vi "Resolve Request State.vi"(7 "status code in":u16, 8 "error in":errorcluster, 9 "response in":string, 10 "refused in":bool, 11 "MCP Request Metadata":T1) -> (0 "error out":errorcluster, 1 "response":string, 2 "refused":bool, 3 "MCP Request Metadata out":T1, 5 "status code":u16)   [LabVIEW 2020, in "MCP Server.lvlib"]
doc: "Resolves the requestState of a modern request (MCP 2026-07-28, multi round-trip requests). Called by Handle MCP Request.vi after Check Modern MCP Request.vi and before Set MCP Request Context.vi, and by Prepare Request Dispatch.vi, so that a refused requestState is answered as a plain HTTP error and never streamed.\n\nWHY: the client sends back only the answers to the LATEST inputRequests, together with the opaque requestState token of the previous input_required result. The answers of the earlier rounds stay in the server (Request State Store.vi) and are merged in here, so a tool that asks several questions in several rounds (Ask User.vi) finds every answer it was given.\n\n- No requestState (request state of MCP Request Metadata.ctl empty), a legacy request, or a request already refused (refused in): everything is passed through unchanged.\n- requestState given: the token is taken from Request State Store.vi. It is refused when it is unknown or expired, or when the method, params.name or the arguments digest (SHA-256 of params.arguments, see Read MCP Request Metadata.vi) differ from the ones it was issued for: refused becomes TRUE, status code 400, response {\"jsonrpc\":\"2.0\",\"id\":<id>,\"error\":{\"code\":-32602,\"message\":\"Invalid params: requestState is unknown, expired or belongs to another request\"}}.\n- Found and matching: input responses of MCP Request Metadata out = the stored answers (\"answers\" of the stored state) merged with the request's inputResponses; the request's value wins for the same key, and keys the tool does not ask for are kept (Ask User.vi ignores them).\n\nThe JSONtext errors are merged and cleared here. error in is passed through unchanged and does not stop the resolution."
uses:
  MCP Server.lvlib
  MCP Request Metadata.ctl
  <vilib>/JDP Science/JSONtext/Next JSON Value.vi
  <vilib>/JDP Science/JSONtext/String Subset.vi
  <vilib>/JDP Science/JSONtext/Parsing/Advance past next JSON Value (inlined COPY).vi
  <vilib>/JDP Science/JSONtext/Parsing/Advance past whitespace.vi
  <vilib>/JDP Science/JSONtext/Parsing/Advance past String.vi
  <vilib>/JDP Science/JSONtext/Parsing/Advance past Number.vi
  <vilib>/JDP Science/JSONtext/Parsing/Advance past Line Ending.vi
  <vilib>/JDP Science/JSONtext/Parsing/Parse Full Path or Item Name.vi
  <vilib>/JDP Science/JSONtext/Parsing/Advance past Array.vi
  <vilib>/JDP Science/JSONtext/Parsing/Advance past Object.vi
  <vilib>/JDP Science/JSONtext/support/Error Cluster From Code.vi
  <vilib>/JDP Science/JSONtext/Offset/Find Item Locations by Path.vi
  <vilib>/JDP Science/JSONtext/Get all Object Items.vi
  <vilib>/JDP Science/JSONtext/Set Multiple Object Items.vi
  <vilib>/JDP Science/JSONtext/JSONtext.lvlib
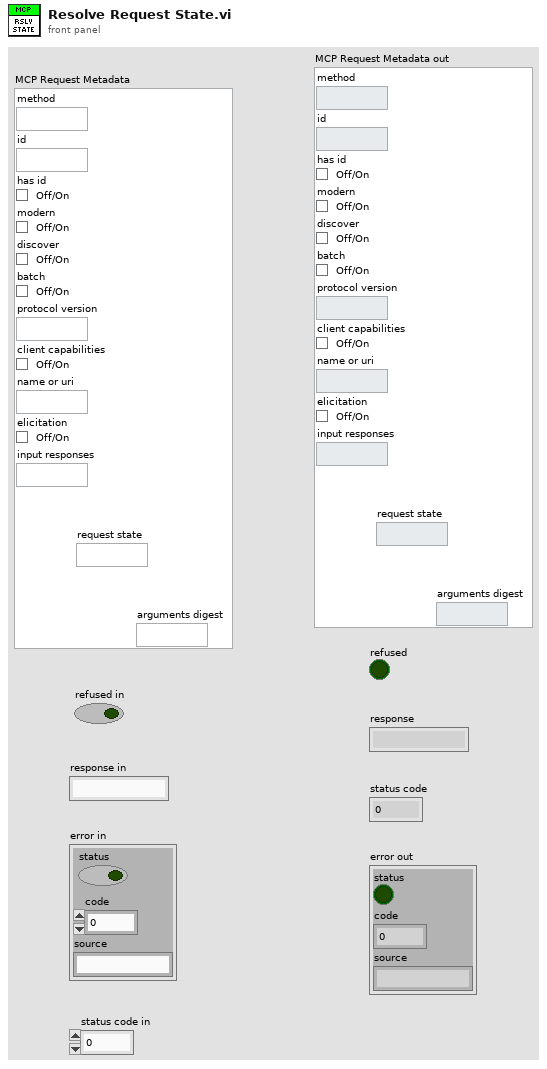
[diagram p1: front panel]
types:
  T1 = typedef "MCP Server.lvlib/MCP Request Metadata.ctl" = cluster{"method":string, "id":string, "has id":bool, "modern":bool, "discover":bool, "batch":bool, "protocol version":string, "client capabilities":bool, "name or uri":string, "elicitation":bool, "input responses":string, "request state":string, "arguments digest":string}
  T2 = cluster{"token":string, "state":string, "method":string, "name":string, "arguments digest":string, "created":u32}
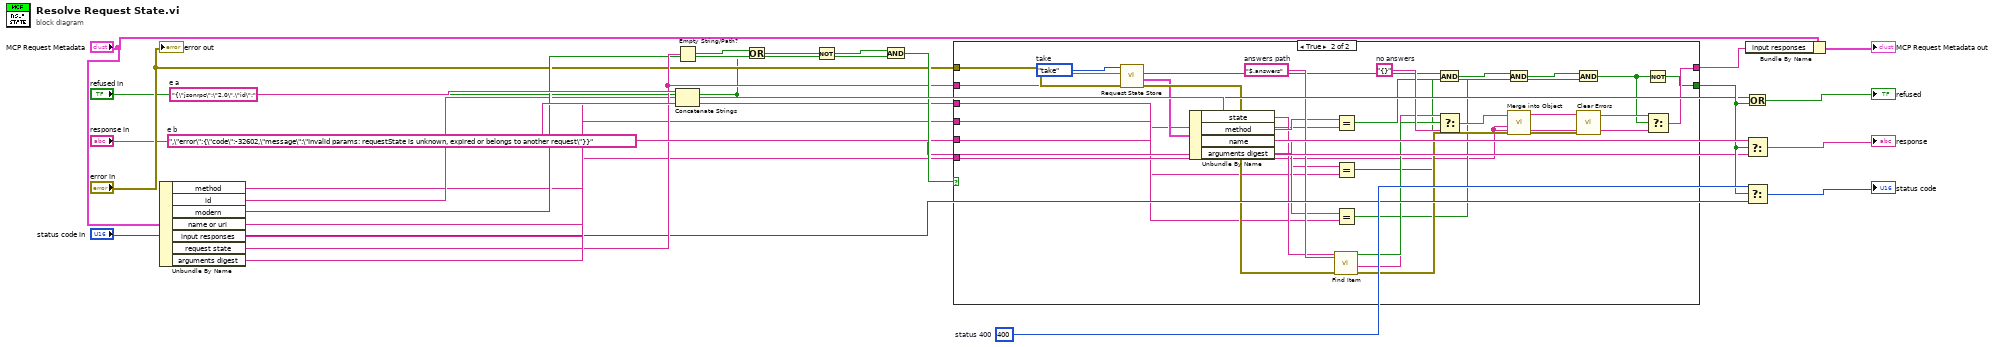
[diagram p0: block diagram]
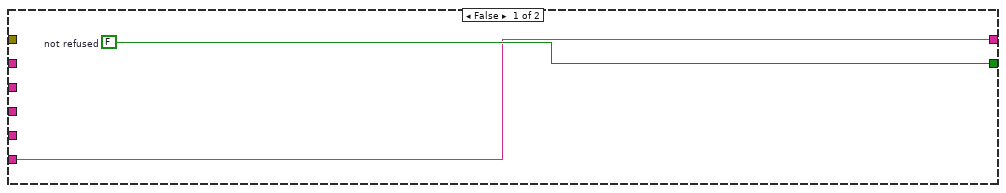
[diagram p2: hidden frame]
diagram:
  w26 = u16 400  # status 400
  w24 = ",\"error\":{\"code\":-32602,\"message\":\"Invalid params: requestState is unknown, expired or belongs to another request\"}}"  # e b
  w23 = "{\"jsonrpc\":\"2.0\",\"id\":"  # e a
  n1 = Unbundle By Name("MCP Request Metadata") -> ("method"=w10:string, "id"=w11:string, "modern"=w12:bool, "name or uri"=w13:string, "input responses"=w14:string, "request state"=w15:string, "arguments digest"=w16:string)
  n2 = Empty String/Path?(string/path=w15) -> (empty?=w17:bool)
  n3 = Concatenate Strings(w23, w11, w24) -> (w25:string)
  n4 = Or(x=w17, y="refused in") -> (x .or. y?=w18:bool)
  n5 = Not(x=w18) -> (.not. x?=w19:bool)
  n6 = And(x=w19, y=w12) -> (x .and. y?=w20:bool)
  n7 = case shown="True" w20 {
    tunnel: "error in" -> [_ w34]
    tunnel: w15 -> [_ w29]
    tunnel: w10 -> [_ w30]
    tunnel: w13 -> [_ w31]
    tunnel: w16 -> [_ w32]
    tunnel: w14 -> [w27 w33]
    tunnel: [w27 w58] -> w21
    tunnel: [w28 w49] -> w22
    frame False {
      w28 = FALSE  # not refused
    }
    frame True {
      w54 = "{}"  # no answers
      w50 = "$.answers"  # answers path
      w35 = enum16{"store", "take", "clear"}."take"  # take
      n8 = call "Request State Store.vi"("error in"=w34, "token"=w29, "action"=w35) -> ("error out"=w38:errorcluster, "entry"=w37:T2, "found?"=w36:bool)  [unwired: 5 in, 1 out]
      n9 = Unbundle By Name(w37) -> ("state"=w39:string, "method"=w40:string, "name"=w41:string, "arguments digest"=w42:string)
      n10 = Equal?(x=w40, y=w30) -> (x = y?=w43:bool)
      n11 = Equal?(x=w41, y=w31) -> (x = y?=w44:bool)
      n12 = Equal?(x=w42, y=w32) -> (x = y?=w45:bool)
      n13 = call <vilib>:"Find Item.vi"("$Path or Item Name"=w50, "error in (no error)"=w38, "JSON"=w39) -> ("error out"=w51:errorcluster, "<JSON>"=w52:string, "Found"=w53:bool)  [unwired: 5 in, 1 out]
      n14 = And(x=w36, y=w43) -> (x .and. y?=w46:bool)
      n15 = Select(t=w52, s=w53, f=w54) -> (s? t:f=w55:string)
      n16 = And(x=w46, y=w44) -> (x .and. y?=w47:bool)
      n17 = call <vilib>:"Merge into Object.vi"("error in (no error)"=w51, "JSON Object to Merge"=w33, "JSON"=w55) -> ("error out"=w57:errorcluster, "<JSON>"=w56:string)  [unwired: 6 in]
      n18 = And(x=w47, y=w45) -> (x .and. y?=w48:bool)
      n19 = call <vilib>:"Clear Errors.vi"("error in (no error)"=w57) -> ()  [unwired: 5 in, 2 out]
      n20 = Not(x=w48) -> (.not. x?=w49:bool)
      n21 = Select(t=w56, s=w48, f=w33) -> (s? t:f=w58:string)
    }
  }
  n22 = Bundle By Name(cluster="MCP Request Metadata", "input responses"=w21) -> (→"MCP Request Metadata out":T1)
  n23 = Or(x="refused in", y=w22) -> (x .or. y?=→"refused":bool)
  n24 = Select(t=w25, s=w22, f="response in") -> (s? t:f=→"response":string)
  n25 = Select(t=w26, s=w22, f="status code in") -> (s? t:f=→"status code":u16)
  "error out" <- "error in"
